vi "Find Changed.vi"(8 "error in (no error)":errorcluster, 10 "Update Objects":T2={"Settings"={"Paths"=[], "Rectangles"=[], "Funnels"=[], "Dots"=[]}, "Data"={"Paths"=[], "Rectangles"=[], "SVGImage"=refnum, "Dots"=[], "Funnels"=[]}}, 11 "Tool Data in":refnum<class "Tool Data.lvclass">) -> (0 "error out":errorcluster, 2 "Changed Objects":T1, 3 "Tool Data out":refnum<class "Tool Data.lvclass">)   [LabVIEW 2019, in "Tool Data.lvclass"]
uses:
  Tool Data.lvclass
  Typedefs/PrivateEvents--Tool Data.Update Objects.ctl
  Parse/Image/SVGImage.lvclass
  Settings/Setting Database/Typedefs/PublicEvents--Setting Database.PathsUpdated.ctl
  Settings/Path Settings/Path Settings.lvclass
  Settings/Setting Database/Typedefs/PublicEvents--Setting Database.RectanglesUpdated.ctl
  Settings/Rectangle Settings/Rectangle Settings.lvclass
  Settings/Setting Database/Typedefs/PublicEvents--Setting Database.FunnelsUpdated.ctl
  Settings/Funnel Settings/Funnel Settings.lvclass
  Settings/Setting Database/Typedefs/PublicEvents--Setting Database.DotsUpdated.ctl
  Settings/Dot Settings/Dot Settings.lvclass
  Parse/ParsePaths/Path.lvclass
  Parse/Rectangle/Rectangle.lvclass
  Parse/Dot/Dot.lvclass
  Tool Data.lvclass/Tool Data.ctl
  Settings/Setting Database/Setting Database.lvclass
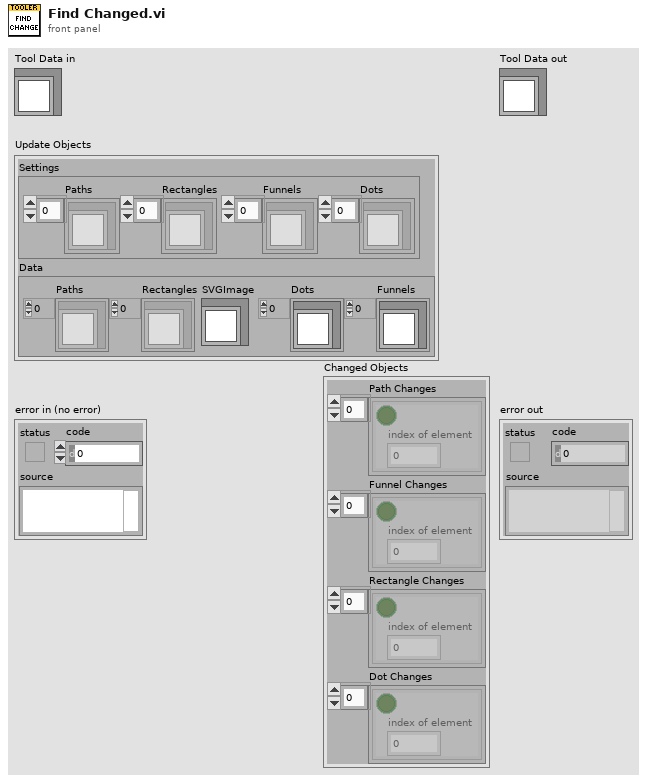
[diagram p1: front panel]
types:
  T1 = cluster{"Path Changes":cluster{bool, "index of element":i32}[], "Funnel Changes":cluster{bool, "index of element":i32}[], "Rectangle Changes":cluster{bool, "index of element":i32}[], "Dot Changes":cluster{bool, "index of element":i32}[]}
  T2 = typedef "Tool Data.lvclass/PrivateEvents--Tool Data.Update Objects.ctl" = cluster{"Settings":cluster{"Paths":T3, "Rectangles":T4, "Funnels":T5, "Dots":T6}, "Data":cluster{"Paths":refnum<class "Path.lvclass">[], "Rectangles":refnum<class "Rectangle.lvclass">[], "SVGImage":refnum<class "SVGImage.lvclass">, "Dots":refnum<class "Dot.lvclass">[], "Funnels":refnum<class "Path.lvclass">[]}}
  T3 = typedef "Setting Database.lvclass/PublicEvents--Setting Database.PathsUpdated.ctl" = refnum<class "Path Settings.lvclass">[]
  T4 = typedef "Setting Database.lvclass/PublicEvents--Setting Database.RectanglesUpdated.ctl" = refnum<class "Rectangle Settings.lvclass">[]
  T5 = typedef "Setting Database.lvclass/PublicEvents--Setting Database.FunnelsUpdated.ctl" = refnum<class "Funnel Settings.lvclass">[]
  T6 = typedef "Setting Database.lvclass/PublicEvents--Setting Database.DotsUpdated.ctl" = refnum<class "Dot Settings.lvclass">[]
  T7 = cluster{"Paths":T3, "Rectangles":T4, "Funnels":T5, "Dots":T6}
  T8 = cluster{"Paths":refnum<class "Path.lvclass">[], "Rectangles":refnum<class "Rectangle.lvclass">[], "SVGImage":refnum<class "SVGImage.lvclass">, "Dots":refnum<class "Dot.lvclass">[], "Funnels":refnum<class "Path.lvclass">[]}
  T9 = cluster{"paths":string[], "funnels":string[], "rects":string[], "dots":string[]}
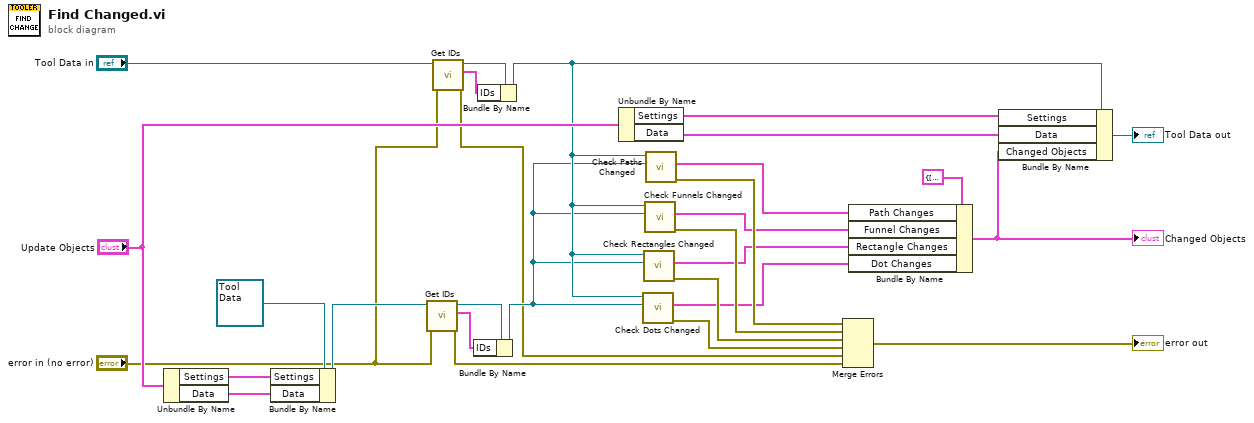
[diagram p0: block diagram]
diagram:
  n1 = Unbundle By Name("Update Objects") -> ("Settings"=w29:T7, "Data"=w28:T8)
  n2 = Bundle By Name(cluster=refnum<class "Tool Data.lvclass"> refnum ("Tool Data in"), "Settings"=w29, "Data"=w28) -> (w20:refnum<class "Tool Data.lvclass">)
  n3 = call "Get IDs.vi"("error in (no error)"="error in (no error)", "Tool Data in"=w20) -> ("error out"=w3:errorcluster, "IDs"=w25:T9, "Tool Data out"=w24:refnum<class "Tool Data.lvclass">)  [unwired: 7 in]
  n4 = call "Get IDs.vi"("error in (no error)"="error in (no error)", "Tool Data in"="Tool Data in") -> ("error out"=w2:errorcluster, "IDs"=w18:T9, "Tool Data out"=w23:refnum<class "Tool Data.lvclass">)  [unwired: 7 in]
  n5 = Bundle By Name(cluster=w24, "IDs"=w25) -> (w4:refnum<class "Tool Data.lvclass">)
  n6 = Bundle By Name(cluster=w23, "IDs"=w18) -> (w8:refnum<class "Tool Data.lvclass">)
  n7 = Unbundle By Name("Update Objects") -> ("Settings"=w6:T7, "Data"=w5:T8)
  n8 = call "Check Dots Changed.vi"("New Tool"=w4, "Tool Data in"=w8) -> ("error out"=w17:errorcluster, "Changed"=w9:cluster{bool, "index of element":i32}[])  [unwired: 7 in, 1 out]
  n9 = call "Check Rectangles Changed.vi"("New Tool"=w4, "Tool Data in"=w8) -> ("error out"=w16:errorcluster, "Changed"=w13:cluster{bool, "index of element":i32}[])  [unwired: 7 in, 1 out]
  n10 = call-dynamic "Check Funnels Changed.vi"("New Tool"=w4, "Tool Data in"=w8) -> ("error out"=w15:errorcluster, "Changed"=w12:cluster{bool, "index of element":i32}[])  [unwired: 7 in, 1 out]
  n11 = call-dynamic "Check Paths Changed.vi"("New Data In"=w4, "Tool Data in"=w8) -> ("error out"=w14:errorcluster, "Changed"=w11:cluster{bool, "index of element":i32}[])  [unwired: 7 in, 1 out]
  n12 = Merge Errors(w14, w15, w16, w17, w2, w3) -> (→"error out":errorcluster)
  n13 = Bundle By Name(cluster=T1 {"Path Changes"=[], "Funnel Changes"=[], "Rectangle Changes"=[], "Dot Changes"=[]}, "Path Changes"=w11, "Funnel Changes"=w12, "Rectangle Changes"=w13, "Dot Changes"=w9) -> (w7:T1)
  "Changed Objects" <- w7
  n14 = Bundle By Name(cluster=w8, "Settings"=w6, "Data"=w5, "Changed Objects"=w7) -> (→"Tool Data out":refnum<class "Tool Data.lvclass">)
